vi "create point buffer.vi"() -> (0 "error out":errorcluster, 3 "point buffer":refnum<data-value>)   [LabVIEW 2020, in "nominal core steps.lvlib"]
doc: "A buffer allowing TestStand to collect individual points and stream them all at once, for efficiency. Intended to represent data for a single channel. Use the batch buffer for many channels."
uses:
  nominal core steps.lvlib
  points buffer.ctl
  single point.ctl
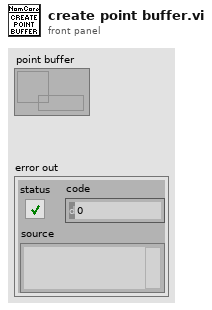
[diagram p1: front panel]
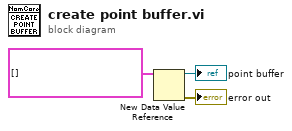
[diagram p0: block diagram]
diagram:
  n1 = New Data Value Reference(data value=cluster{"Time Stamp":timestamp, "Value":dbl}[] [] ("Points")) -> (data value reference=→"point buffer":refnum<data-value>, error out=→"error out":errorcluster)  [unwired: 1 in]
